vi "Delete Platform Application.vi"(8 "error in (no error)":errorcluster, 11 "Platform Application in":refnum<class "Platform Application.lvclass">) -> (0 "error out":errorcluster)   [LabVIEW 2015, in "NI_AWS_SNS.lvlib" / "Platform Application.lvclass"]
doc: "Deletes a platform application object for one of the supported push notification services, such as APNS and GCM."
uses:
  Platform Application.lvclass
  Core/ARN/ARN.lvclass
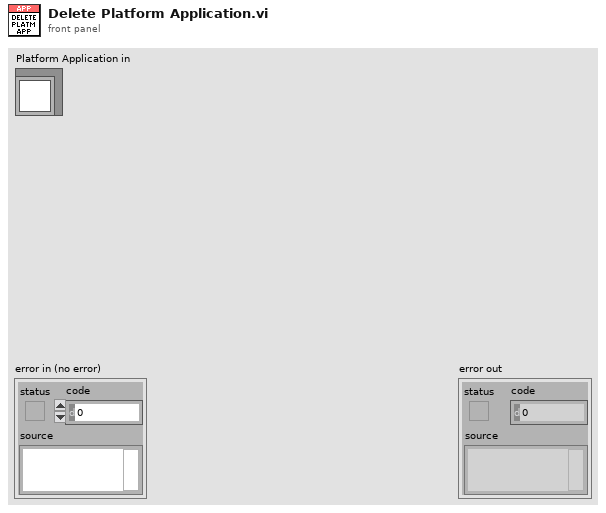
[diagram p1: front panel]
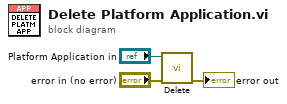
[diagram p0: block diagram]
diagram:
  n1 = call "Delete.vi"("error in (no error)"="error in (no error)", "ARN in"="Platform Application in") -> ("error out"=→"error out":errorcluster)  [unwired: 9 in]
